vi "Sous_VI_RT_recule.vi"(8 "Erreur IN":errorcluster caption="Erreur", 10 "Compteur IN":i32, 11 "Etat IN":T1) -> (0 "Erreur OUT":errorcluster caption="Erreur", 1 "Indicateur fin de process":bool, 2 "Compteur OUT":i32, 3 "Etat OUT":T1, 5 "Detection suiveur de ligne":bool[](array[boolean]))   [LabVIEW 2018]
doc: "fait légèrement avancer le robot avant de le faire reculer"
uses:
  enum_RT_recule.ctl
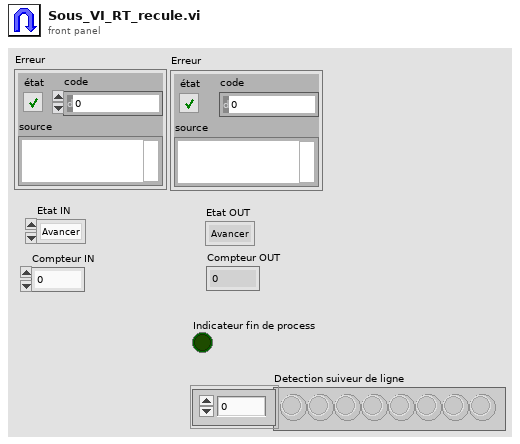
[diagram p1: front panel]
types:
  T1 = typedef "enum_RT_recule.ctl" = enum16{"Avancer", "Reculer", "STOP"}
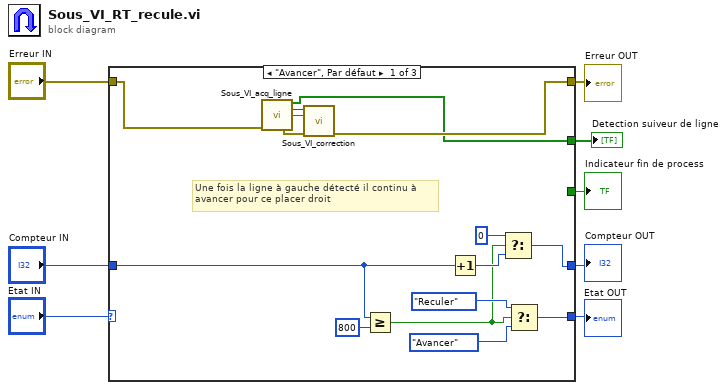
[diagram p0: block diagram]
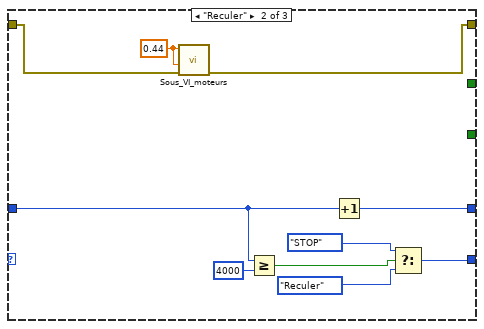
[diagram p2: hidden frame]
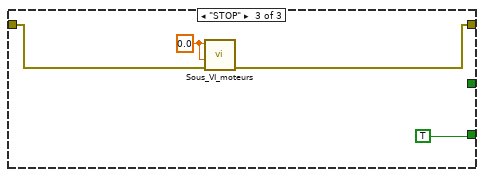
[diagram p3: hidden frame]
diagram:
  n1 = case shown="\"Avancer\", Par défaut" "Etat IN" {
    tunnel: "Erreur IN" -> [w20 w32 w36]
    tunnel: [w19 w31 w35] -> w8
    tunnel: [w18 w26 _] -> w3
    tunnel: [w12 w28 _] -> w5
    tunnel: "Compteur IN" -> [w16 w27 _]
    tunnel: [_ _ TRUE] -> w2
    tunnel: [w13 _ _] -> w1
    frame "Avancer", Default {
      # "Une fois la ligne à gauche détecté il continu à \navancer pour ce placer droit"
      n2 = call "Sous_VI_acq_ligne.vi"("error in (no error)"=w20) -> ("x > y ?"=w13:bool[], "Décalage"=w23:u32, "G/D ?"=w22:bool, "error out"=w21:errorcluster)  [unwired: 9 in, 2 out]
      n3 = call "Sous_VI_correction.vi"("error in (no error)"=w21, "G/D ?"=w22, "Décalage"=w23) -> ("error out"=w19:errorcluster)  [unwired: 8 in]
      n4 = Greater Or Equal?(x=w16, y=800) -> (x >= y?=w9:bool)
      n5 = Increment(x=w16) -> (x+1=w11:i32)
      n6 = Select(t=0 ("cas vrai"), s=w9, f=w11) -> (s? t:f=w12:i32)
      n7 = Select(t=enum_RT_recule."Reculer", s=w9, f=enum_RT_recule."Avancer") -> (s? t:f=w18:T1)
    }
    frame "Reculer" {
      w33 = 0.44 ("moteur gauche vite")
      n8 = call "Sous_VI_moteurs.vi"("error in (no error)"=w32, "Moteur Droit"=w33, "Moteur Gauche"=w33) -> ("error out"=w31:errorcluster)  [unwired: 8 in]
      n9 = Greater Or Equal?(x=w27, y=4000) -> (x >= y?=w29:bool)
      n10 = Increment(x=w27) -> (x+1=w28:i32)
      n11 = Select(t=enum_RT_recule."STOP", s=w29, f=enum_RT_recule."Reculer") -> (s? t:f=w26:T1)
    }
    frame "STOP" {
      w37 = 0.0 ("Moteur Gauche")
      n12 = call "Sous_VI_moteurs.vi"("error in (no error)"=w36, "Moteur Droit"=w37, "Moteur Gauche"=w37) -> ("error out"=w35:errorcluster)  [unwired: 8 in]
    }
  }
  "Erreur OUT" <- w8
  "Compteur OUT" <- w5
  "Etat OUT" <- w3
  "Indicateur fin de process" <- w2
  "Detection suiveur de ligne" <- w1
